vi "update Graph.vi"(0 "GrphChrt Ref In":refnum<vi>, 5 "Interpret as Unicode (T)":bool=TRUE, 7 "X Axis Label":string[](array[string]), 9 "Y Axis Label":string[](array[string]), 11 "error in (no error)":errorcluster) -> (4 "GrphChrt Ref Out":refnum<vi>, 15 "error out":errorcluster)   [LabVIEW 2019, in "Language Selection.lvlib"]
doc: "Uses \"X Axis Label\" and \"Y Axis Label\" input strings to translate the labels of a Graph/Chart control.\n- - -\nCopyright (c) 2026, Merecs Engineering GmbH"
uses:
  Language Selection.lvlib
panel:
  # "Connector Pane"
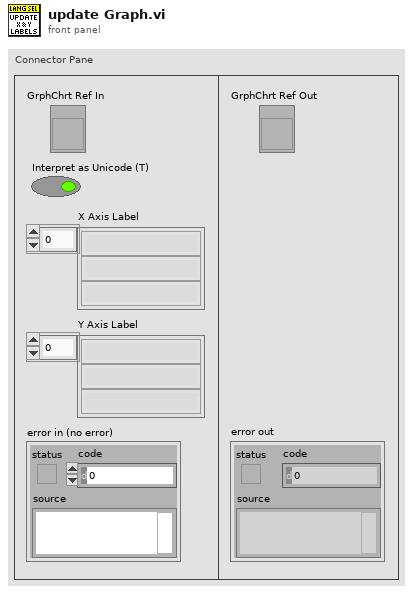
[diagram p1: front panel]
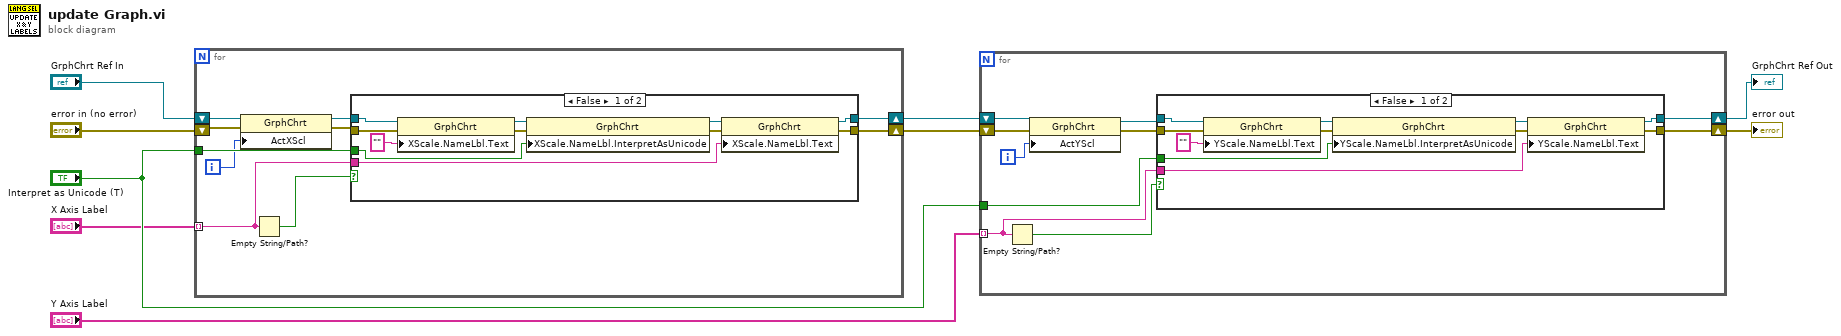
[diagram p0: block diagram]
diagram:
  n1 = for {
    tunnel: "Interpret as Unicode (T)" -> [w16]
    tunnel: "X Axis Label" -> [w14] mode=indexing
    shift-right: [w19] -> w9
    shift-left: "GrphChrt Ref In" -> [w15]
    shift-right: [w17] -> w8
    shift-left: "error in (no error)" -> [w12]
    i -> [w10]
    n2 = property class="GrphChrt"(reference=w15, error in=w12, "ActXScl"=w10) -> (reference out=w13:refnum<vi>, error out=w11:errorcluster)
    n3 = Empty String/Path?(string/path=w14) -> (empty?=w18:bool)
    n4 = case shown="False" w18 {
      tunnel: w13 -> [w25 w32]
      tunnel: [w23 w32] -> w19
      tunnel: w16 -> [w22 _]
      tunnel: [w24 w31] -> w17
      tunnel: w14 -> [w21 _]
      tunnel: w11 -> [w20 w31]
      frame False {
        n5 = property class="GrphChrt"(reference=w25, error in=w20, "XScale.NameLbl.Text"="" ("Caption.Text")) -> (reference out=w26:refnum<vi>, error out=w27:errorcluster)
        n6 = property class="GrphChrt"(reference=w26, error in=w27, "XScale.NameLbl.InterpretAsUnicode"=w22) -> (reference out=w29:refnum<vi>, error out=w30:errorcluster)
        n7 = property class="GrphChrt"(reference=w29, error in=w30, "XScale.NameLbl.Text"=w21) -> (reference out=w23:refnum<vi>, error out=w24:errorcluster)
      }
      frame True {
      }
    }
  }
  n8 = for {
    tunnel: "Interpret as Unicode (T)" -> [w38]
    tunnel: "Y Axis Label" -> [w37] mode=indexing
    shift-right: [w39] -> w6
    shift-left: w9 -> [w35]
    shift-right: [w40] -> w7
    shift-left: w8 -> [w41]
    i -> [w33]
    n9 = Empty String/Path?(string/path=w37) -> (empty?=w42:bool)
    n10 = property class="GrphChrt"(reference=w35, error in=w41, "ActYScl"=w33) -> (reference out=w34:refnum<vi>, error out=w36:errorcluster)
    n11 = case shown="False" w42 {
      tunnel: [w44 w55] -> w40
      tunnel: w36 -> [w47 w55]
      tunnel: w34 -> [w46 w54]
      tunnel: w38 -> [w48 _]
      tunnel: [w45 w54] -> w39
      tunnel: w37 -> [w43 _]
      frame False {
        n12 = property class="GrphChrt"(reference=w46, error in=w47, "YScale.NameLbl.Text"="" ("Caption.Text")) -> (reference out=w49:refnum<vi>, error out=w50:errorcluster)
        n13 = property class="GrphChrt"(reference=w49, error in=w50, "YScale.NameLbl.InterpretAsUnicode"=w48) -> (reference out=w52:refnum<vi>, error out=w53:errorcluster)
        n14 = property class="GrphChrt"(reference=w52, error in=w53, "YScale.NameLbl.Text"=w43) -> (reference out=w45:refnum<vi>, error out=w44:errorcluster)
      }
      frame True {
      }
    }
  }
  "error out" <- w7
  "GrphChrt Ref Out" <- w6
